vi "Create Map of Parameter Names.vi"(8 "error in (no error)":errorcluster, 11 "Kasli in":refnum<class "Kasli.lvclass">) -> (0 "error out":errorcluster, 2 "Parameters Map":map{string, string[]}(c390), 3 "Kasli out":refnum<class "Kasli.lvclass">)   [LabVIEW 2020, in "Kasli Wrapper 2.0.lvlib" / "Kasli.lvclass"]
doc: "This VI reads the Build and Init.py library and retrieves the mapping of Kasli names to the list of parameters for the script"
uses:
  Kasli.lvclass
  Kasli.lvclass/Kasli.ctl
  <vilib>/Utility/error.llb/whitespace.ctl
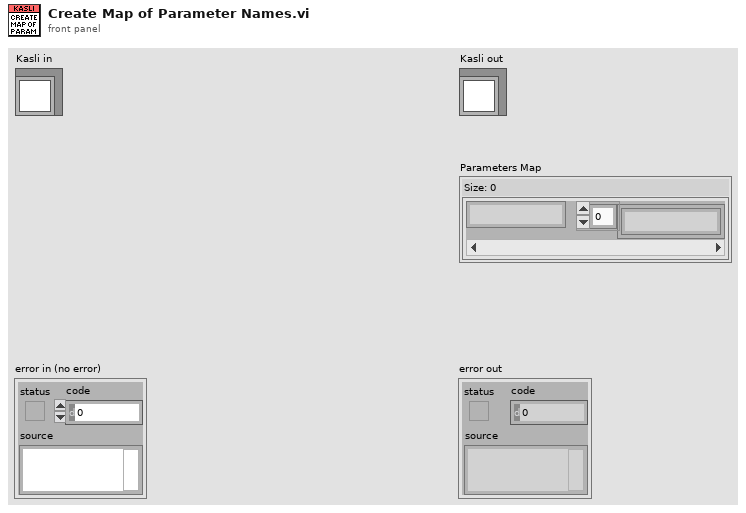
[diagram p1: front panel]
types:
  T1 = typedef "whitespace.ctl" = u16
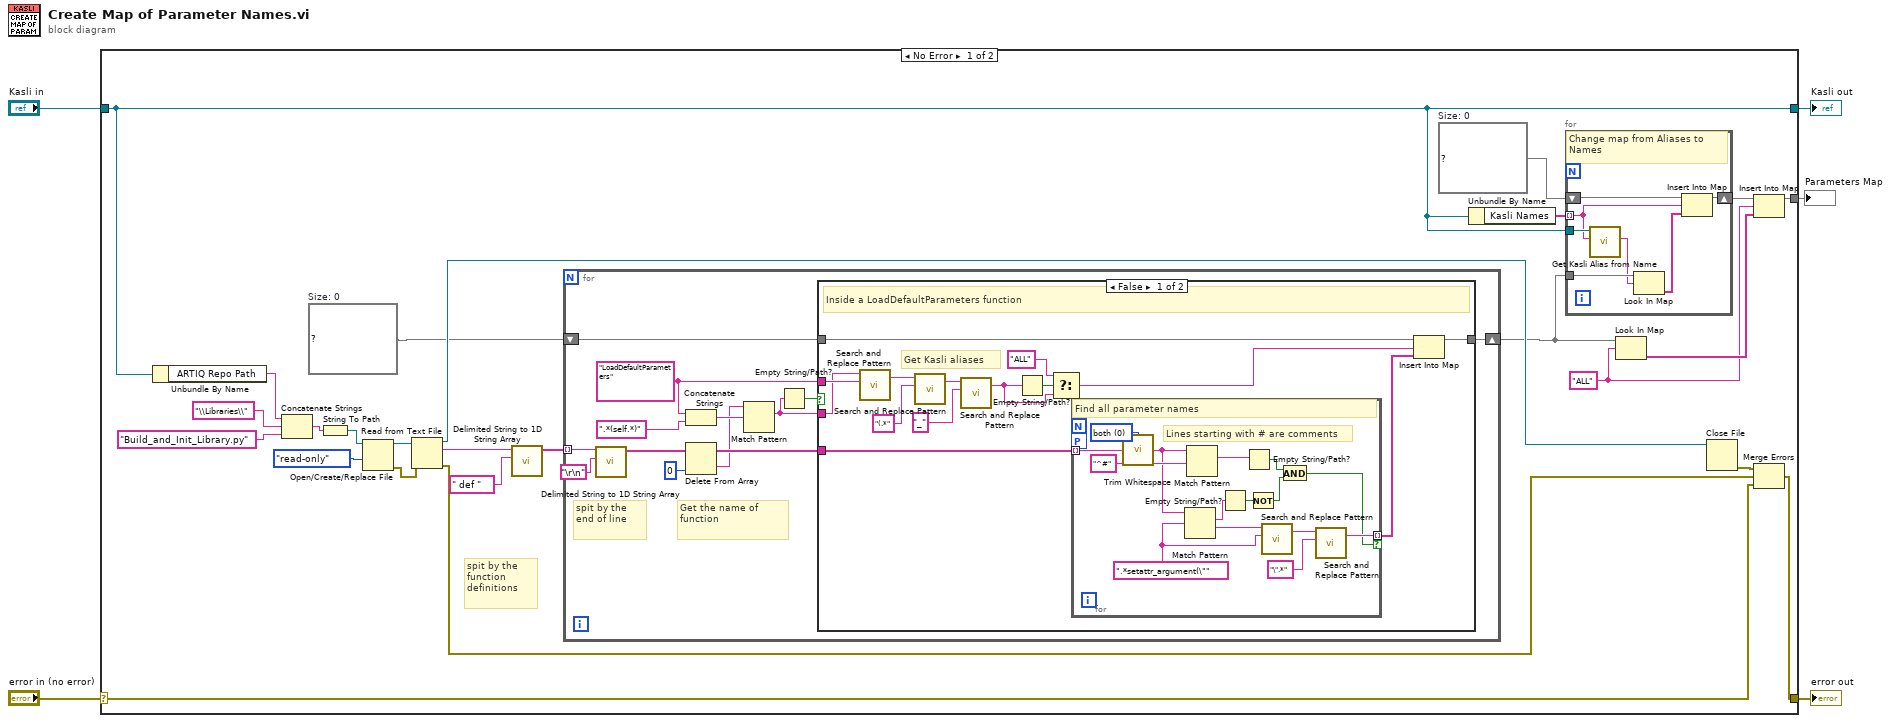
[diagram p0: block diagram]
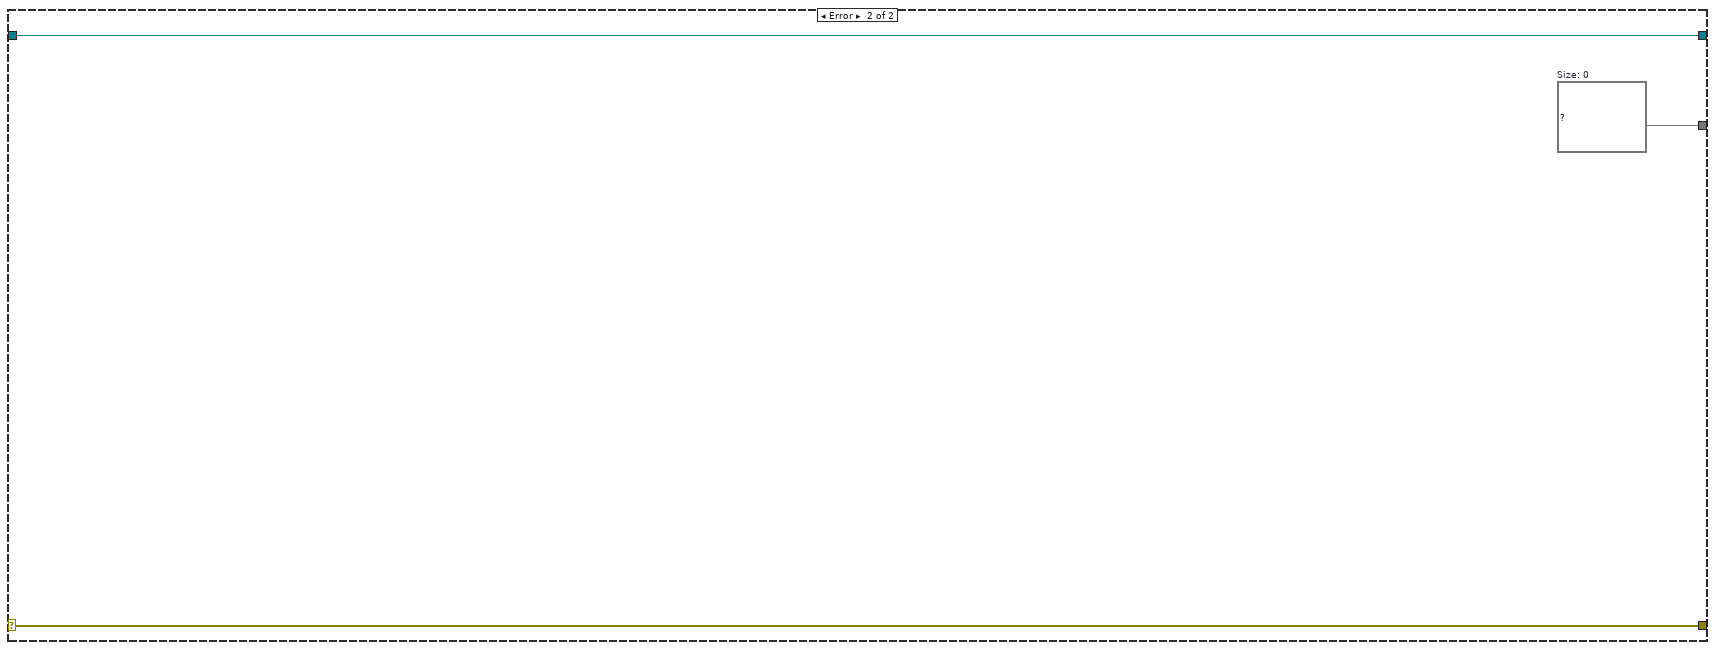
[diagram p3: hidden frame]
diagram:
  n1 = case shown="No Error" "error in (no error)" {
    selector: "error in (no error)" -> [w17 w83]
    tunnel: [w16 w83] -> w4
    tunnel: [w13 w82] -> w2
    tunnel: "Kasli in" -> [w13 w82]
    tunnel: [w12 w81] -> w1
    frame No Error {
      w9 = "ALL" ("key")
      w14 = map{string, string[]} {}  # Size: 0
      w26 = map{string, string[]} {}  # Size: 0
      # "spit by the function definitions"
      n2 = Unbundle By Name(w13) -> ("ARTIQ Repo Path"=w19:string)
      n3 = Concatenate Strings(w19, "\\Libraries\\" ("string"), "Build_and_Init_Library.py") -> (w22:string)
      n4 = String To Path(string=w22) -> (path=w21:path)
      n5 = Open/Create/Replace File(file path (use dialog)=w21, access (0:read/write)=enum16{"read/write", "read-only", "write-only"}."read-only") -> (refnum out=w29:refnum<file>, error out=w18:errorcluster)  [unwired: 4 in, 1 out]
      n6 = Read from Text File(file (use dialog)=w29, error in=w18) -> (refnum out=w28:refnum<file>, text=w7:string, error out=w25:errorcluster)  [unwired: 2 in, 1 out]
      n7 = call <vilib>:"Delimited String to 1D String Array.vi"("delimiter"=" def ", "delimited string"=w7) -> ("string array"=w8:string[])  [unwired: 9 in]
      n8 = for {
        tunnel: w8 -> [w43] mode=indexing
        shift-right: [w32] -> w10
        shift-left: w26 -> [w33]
        w40 = "LoadDefaultParameters" ("regular expression")
        # "Get the name of function"
        # "spit by the end of line"
        n9 = call <vilib>:"Delimited String to 1D String Array.vi"("delimiter"="\r\n", "delimited string"=w43) -> ("string array"=w38:string[])  [unwired: 9 in]
        n10 = Concatenate Strings(w40, ".*(self.*)" ("regular expression")) -> (w41:string)
        n11 = Delete From Array(array=w38, index=0) -> (deleted portion=w36:string, array with subset deleted=w37:string[])  [unwired: 1 in]
        n12 = Match Pattern(string=w36, regular expression=w41) -> (match substring=w35:string)  [unwired: 1 in, 3 out]
        n13 = Empty String/Path?(string/path=w35) -> (empty?=w34:bool)
        n14 = case shown="False" w34 {
          tunnel: w40 -> [w57 _]
          tunnel: w37 -> [w50 _]
          tunnel: w35 -> [w49 _]
          tunnel: w33 -> [w47 w73]
          tunnel: [w48 w73] -> w32
          frame False {
            # "Get Kasli aliases"
            # "Inside a LoadDefaultParameters function"
            n15 = call <vilib>:"Search and Replace Pattern.vi"("string"=w49, "regular expression (\"\")"=w57) -> ("result string"=w56:string)  [unwired: 3 in, 1 out]
            n16 = call <vilib>:"Search and Replace Pattern.vi"("string"=w56, "regular expression (\"\")"="(.*" ("regular expression (\"\")")) -> ("result string"=w54:string)  [unwired: 3 in, 1 out]
            n17 = call <vilib>:"Search and Replace Pattern.vi"("string"=w54, "regular expression (\"\")"="_" ("search string")) -> ("result string"=w52:string)  [unwired: 3 in, 1 out]
            n18 = Empty String/Path?(string/path=w52) -> (empty?=w53:bool)
            n19 = Select(t="ALL", s=w53, f=w52) -> (s? t:f=w45:string)
            n20 = for {
              tunnel: w50 -> [w69] mode=indexing
              tunnel: [w66] -> w46 mode=indexing if=w62
              workers-P: _ -> [_]
              w72 = T1 0 items=["both", "start of string", "end of string"] ("location (both)")
              w67 = ".*setattr_argument(\""
              # "Lines starting with # are comments"
              # "Find all parameter names"
              n21 = call <vilib>:"Trim Whitespace.vi"("string"=w69, "location (both)"=w72) -> ("trimmed string"=w68:string)
              n22 = Match Pattern(string=w68, regular expression=w67) -> (match substring=w64:string, after substring=w71:string)  [unwired: 1 in, 2 out]
              n23 = Match Pattern(string=w68, regular expression="^#") -> (match substring=w65:string)  [unwired: 1 in, 3 out]
              n24 = Empty String/Path?(string/path=w64) -> (empty?=w61:bool)
              n25 = Empty String/Path?(string/path=w65) -> (empty?=w63:bool)
              n26 = Not(x=w61) -> (.not. x?=w60:bool)
              n27 = call <vilib>:"Search and Replace Pattern.vi"("string"=w71, "regular expression (\"\")"=w67) -> ("result string"=w59:string)  [unwired: 3 in, 1 out]
              n28 = And(x=w63, y=w60) -> (x .and. y?=w62:bool)
              n29 = call <vilib>:"Search and Replace Pattern.vi"("string"=w59, "regular expression (\"\")"="\".*" ("regular expression (\"\")")) -> ("result string"=w66:string)  [unwired: 3 in, 1 out]
            }
            n30 = Insert Into Map(map in=w47, key=w45, value=w46) -> (map out=w48:map{string, string[]})  [unwired: 2 out]
          }
          frame True {
            # "Not a LoadDefaultParameters function, ignore"
          }
        }
      }
      n31 = Unbundle By Name(w13) -> ("Kasli Names"=w15:string[])
      n32 = for {
        tunnel: w15 -> [w76] mode=indexing
        shift-right: [w79] -> w11
        shift-left: w14 -> [w80]
        tunnel: w10 -> [w78]
        tunnel: w13 -> [w77]
        # "Change map from Aliases to Names"
        n33 = call-dynamic "Get Kasli Alias from Name.vi"("Kasli Name"=w76, "Kasli in"=w77) -> ("Kasli Alias"=w75:string)  [unwired: 7 in, 2 out]
        n34 = Look In Map(map=w78, key=w75) -> (value=w74:string[])  [unwired: 1 in, 1 out]
        n35 = Insert Into Map(map in=w80, key=w76, value=w74) -> (map out=w79:map{string, string[]})  [unwired: 2 out]
      }
      n36 = Look In Map(map=w10, key=w9) -> (value=w30:string[])  [unwired: 1 in, 1 out]
      n37 = Close File(refnum=w28) -> (error out=w24:errorcluster)  [unwired: 1 in, 1 out]
      n38 = Insert Into Map(map in=w11, key=w9, value=w30) -> (map out=w12:map{string, string[]})  [unwired: 2 out]
      n39 = Merge Errors(w24, w25, w17) -> (w16:errorcluster)
    }
    frame Error {
      w81 = map{string, string[]} {}  # Size: 0
    }
  }
  "error out" <- w4
  "Kasli out" <- w2
  "Parameters Map" <- w1
